vi "Host_Main.vi"(8 "error in (no error)":errorcluster={"status"=FALSE, "code"=0, "source"="\"\""}, 10 "application path":string="app_path", 11 "Startup config":string="config.json") -> (0 "error out":errorcluster={"status"=FALSE, "code"=0, "source"="\"\""}, 2 "status ok":bool, 3 "Stop status":string)   [LabVIEW 2026]
doc: "INTENT: Top-level Host Application Entry orchestrating Event Handling Loop (Producer) and Message Handling Loop (Consumer)."
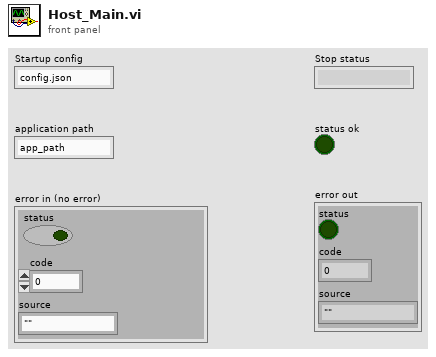
[diagram p1: front panel]
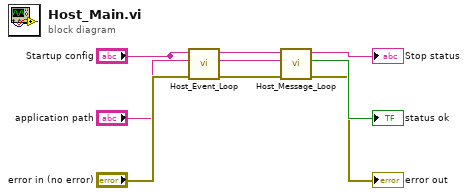
[diagram p0: block diagram]
diagram:
  n1 = call "Host_Event_Loop.vi"("error in (no error)"="error in (no error)", "event loop queue"="application path", "UI references"="Startup config") -> ("error out"=w5:errorcluster, "Host messages"=w4:string)  [unwired: 6 in, 1 out]
  n2 = call "Host_Message_Loop.vi"("error in (no error)"=w5, "app-state shift register"="Startup config", "HostMessage.ctl queue"=w4) -> ("error out"=→"error out":errorcluster, "status ok"=→"status ok":bool, "HMI updates"=→"Stop status":string)  [unwired: 6 in]
